vi "TDMS_Make_Path.vi"(0 "Save Folder":path, 11 "error in":errorcluster) -> (4 "File Path":path, 15 "error out":errorcluster)   [LabVIEW 2026]
doc: "저장 폴더 + AI_YYYYMMDD_HHMMSS.tdms 경로 생성."
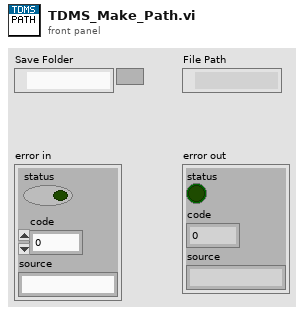
[diagram p1: front panel]
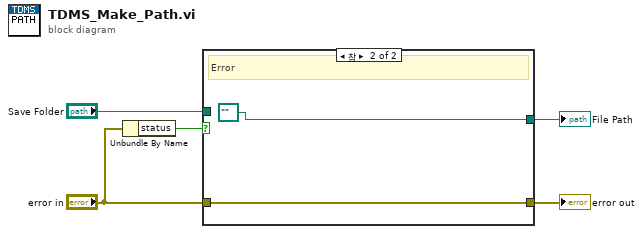
[diagram p0: block diagram]
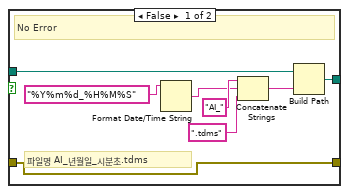
[diagram p2: hidden frame]
diagram:
  n1 = Unbundle By Name("error in") -> ("status"=w3:bool)
  n2 = case shown="참" w3 {
    tunnel: "Save Folder" -> [w6 _]
    tunnel: "error in" -> [w7 w14]
    tunnel: [w7 w14] -> w5
    tunnel: [w13 path ""] -> w4
    frame False {
      # "파일명 AI_년월일_시분초.tdms"
      # "No Error"
      n3 = Format Date/Time String(time format string (%c)="%Y%m%d_%H%M%S") -> (date/time string=w9:string)  [unwired: 1 in, 1 out]
      n4 = Concatenate Strings("AI_", w9, ".tdms") -> (w12:string)
      n5 = Build Path(base path=w6, name or relative path=w12) -> (appended path=w13:path)
    }
    frame True {
      # "Error"
    }
  }
  "File Path" <- w4
  "error out" <- w5
